vi "ReadVamp.vi"() -> ()   [LabVIEW 2015]
panel:
  in  "VISA资源名称":refnum<visa-resource-name>
  out "幅度值":string
  in  "时基(s)":string="0.0005"
  in  "垂直挡位(V)":string="0.5"
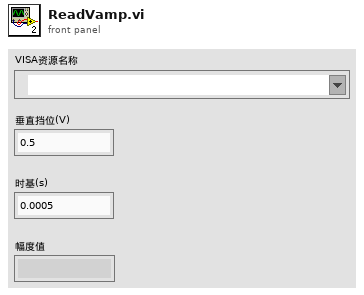
[diagram p1: front panel]
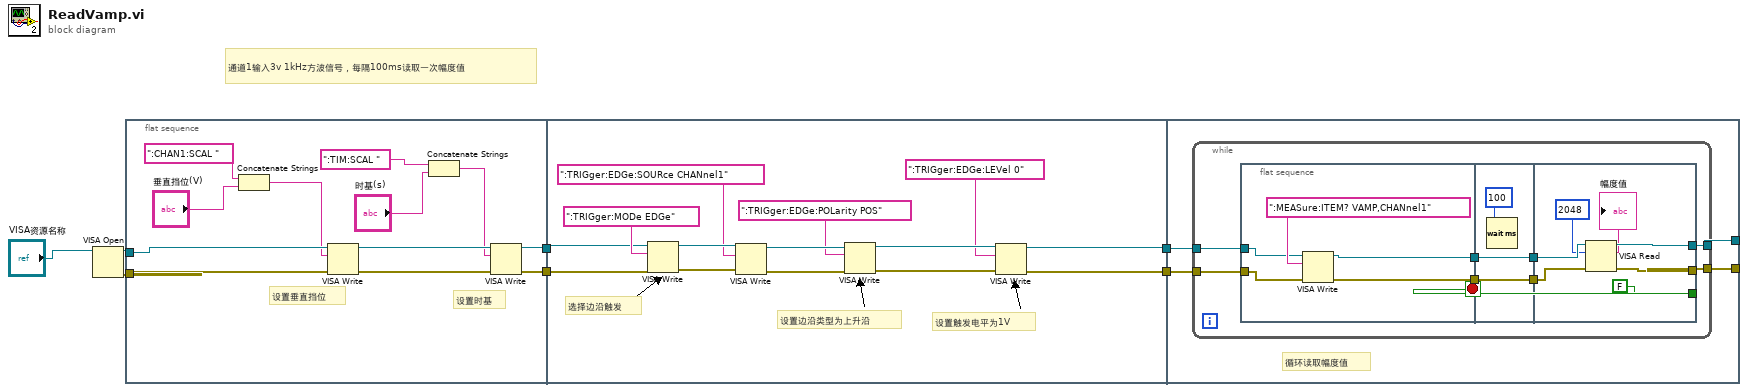
[diagram p0: block diagram]
diagram:
  # "通道1输入3v 1kHz方波信号，每隔100ms读取一次幅度值"
  n1 = VISA Open(VISA resource name="VISA资源名称") -> (VISA resource name=w7:refnum<visa-resource-name>, error out=w6:errorcluster)  [unwired: 4 in]
  n2 = flat-sequence {
    tunnel: w7 -> [w18]
    tunnel: w6 -> [w10]
    tunnel: [w9] -> w4
    tunnel: [w8] -> w2
    tunnel: w4 -> [w22]
    tunnel: [w21] -> w3
    tunnel: w2 -> [w23]
    tunnel: [w20] -> w1
    tunnel: [w37] -> _
    tunnel: [w36] -> _
    tunnel: w3 -> [w35]
    tunnel: w1 -> [w34]
    frame #0 {
      # "设置时基"
      # "设置垂直挡位"
      n3 = Concatenate Strings(":CHAN1:SCAL ", "垂直挡位(V)") -> (w17:string)
      n4 = VISA Write(VISA resource name=w18, write buffer=w17, error in (no error)=w10) -> (VISA resource name out=w15:refnum<visa-resource-name>, error out=w11:errorcluster)  [unwired: 1 out]
      n5 = Concatenate Strings(":TIM:SCAL ", "时基(s)") -> (w12:string)
      n6 = VISA Write(VISA resource name=w15, write buffer=w12, error in (no error)=w11) -> (VISA resource name out=w9:refnum<visa-resource-name>, error out=w8:errorcluster)  [unwired: 1 out]
    }
    frame #1 {
      # "设置触发电平为1V"
      # "设置边沿类型为上升沿"
      # "选择边沿触发"
      n7 = VISA Write(VISA resource name=w22, write buffer=":TRIGger:MODe EDGe", error in (no error)=w23) -> (VISA resource name out=w32:refnum<visa-resource-name>, error out=w30:errorcluster)  [unwired: 1 out]
      n8 = VISA Write(VISA resource name=w32, write buffer=":TRIGger:EDGe:SOURce CHANnel1" ("写入缓冲区"), error in (no error)=w30) -> (VISA resource name out=w31:refnum<visa-resource-name>, error out=w29:errorcluster)  [unwired: 1 out]
      n9 = VISA Write(VISA resource name=w31, write buffer=":TRIGger:EDGe:POLarity POS" ("写入缓冲区"), error in (no error)=w29) -> (VISA resource name out=w26:refnum<visa-resource-name>, error out=w25:errorcluster)  [unwired: 1 out]
      n10 = VISA Write(VISA resource name=w26, write buffer=":TRIGger:EDGe:LEVel 0" ("写入缓冲区"), error in (no error)=w25) -> (VISA resource name out=w21:refnum<visa-resource-name>, error out=w20:errorcluster)  [unwired: 1 out]
    }
    frame #2 {
      # "循环读取幅度值"
      n11 = while {
        tunnel: [w41] -> w37
        tunnel: [w40] -> w36
        tunnel: w35 -> [w39]
        tunnel: w34 -> [w38]
        stop <- w45 stop-if-true
        n12 = flat-sequence {
          tunnel: [w51] -> w44
          tunnel: [w49] -> w43
          tunnel: w39 -> [w48]
          tunnel: w38 -> [w47]
          tunnel: [w54] -> w46
          tunnel: w44 -> [w54]
          tunnel: w43 -> [w52]
          tunnel: [w52] -> w42
          tunnel: w46 -> [w61]
          tunnel: [w60] -> w40
          tunnel: [FALSE] -> w45
          tunnel: w42 -> [w57]
          tunnel: [w56] -> _
          tunnel: [w56] -> w41
          frame #0 {
            n13 = VISA Write(VISA resource name=w48, write buffer=":MEASure:ITEM? VAMP,CHANnel1", error in (no error)=w47) -> (VISA resource name out=w51:refnum<visa-resource-name>, error out=w49:errorcluster)  [unwired: 1 out]
          }
          frame #1 {
            n14 = Wait (ms)(milliseconds to wait=100) -> ()  [unwired: 1 out]
          }
          frame #2 {
            n15 = VISA Read(VISA resource name=w61, byte count=2048, error in (no error)=w57) -> (VISA resource name out=w60:refnum<visa-resource-name>, read buffer=→"幅度值":string, error out=w56:errorcluster)  [unwired: 1 out]
          }
        }
      }
    }
  }
